vi "GetXPos.vi"(7 "Menu":refnum<class "Menu.lvclass">, 9 "SubMenu":bool[](array[boolean]), 10 "Array":T1[](array[typedef]), 11 "Item Names":string[](array[string])) -> (1 "ShortCut Text":string[](array[string]), 2 "Start ShortCut":i16, 3 "Total X":i16)   [LabVIEW 2021, in "Menu.lvlib" / "Menu.lvclass"]
uses:
  Menu.lvclass
  <vilib>/Utility/miscctls.llb/LVMenuShortCut.ctl
  Picture2D/src/Text/Text.lvclass
  C:/GitHub/Picture2D/src/IDrawable/IDrawable.lvclass
  C:/GitHub/Picture2D/src/Picture2D/Picture2D.lvclass
  Picture2D/src/2DPictureControl/2DPictureControl.lvclass
  Picture2D/src/Color/Color.lvclass
  Picture2D/src/Collection/Collection.lvclass
  Picture2D/src/Point/Point.lvclass
  GetFont.vi
  GetDesiredFont.vi
  Picture2D/src/Font/Font.lvclass
panel:
  out "2D Picture out":picture
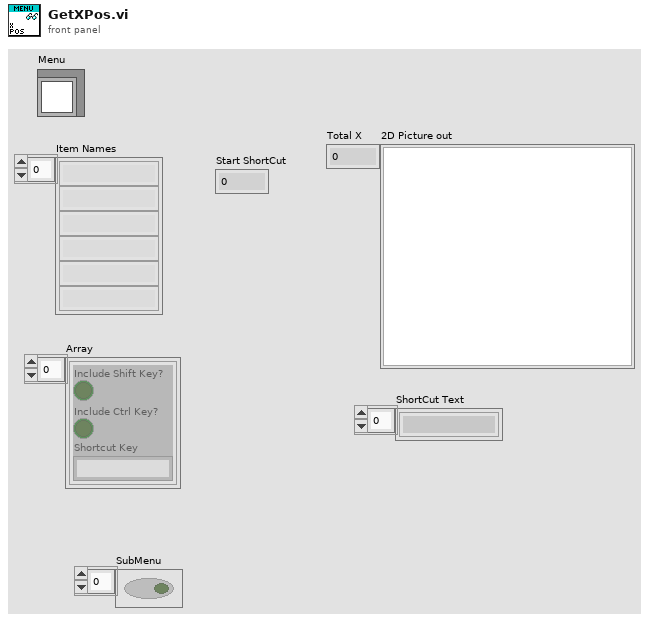
[diagram p1: front panel]
types:
  T1 = typedef "LVMenuShortCut.ctl" = cluster{"Include Shift Key?":bool, "Include Ctrl Key?":bool, "Shortcut Key":string}
  T2 = enum16{"User-specified Font", "Application Font", "System Font", "Dialog Font"}
  T3 = cluster{"left":i16, "top":i16, "right":i16, "bottom":i16}
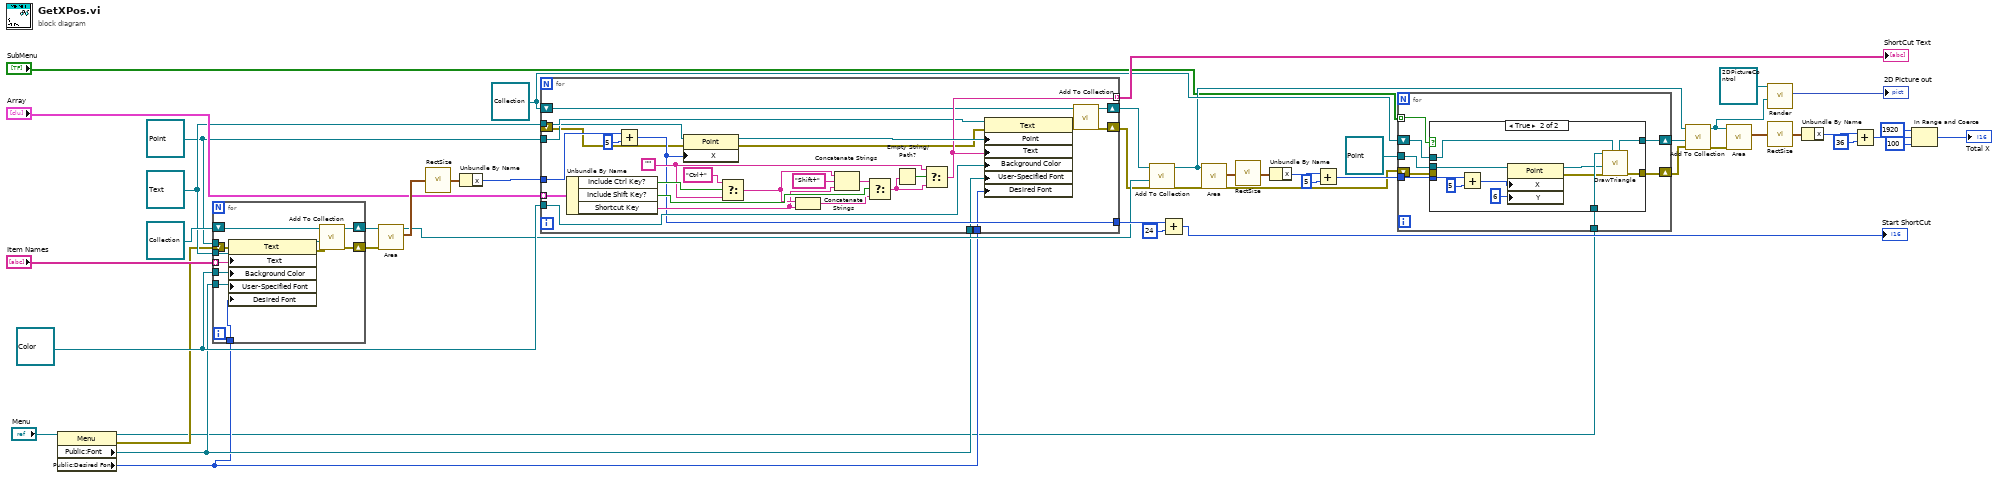
[diagram p0: block diagram]
diagram:
  w27 = refnum<class "Collection.lvclass"> refnum ("Picture2D.lvlib:Collection.lvclass")
  w34 = refnum<class "Color.lvclass"> refnum ("Color")
  w35 = refnum<class "Point.lvclass"> refnum ("Point")
  w36 = refnum<class "Text.lvclass"> refnum ("Text in")
  n1 = property class="Menu"(reference="Menu") -> (reference out=w1:refnum<class "Menu.lvclass">, error out=w2:errorcluster, "Public:Font"=w4:refnum<class "Font.lvclass">, "Public:Desired Font"=w3:T2)  [unwired: 1 in]
  n2 = for {
    tunnel: w36 -> [w56]
    tunnel: "Item Names" -> [w57] mode=indexing
    shift-right: [w58] -> w46
    shift-left: refnum<class "Collection.lvclass"> refnum ("Picture2D.lvlib:Collection.lvclass") -> [w59]
    tunnel: w35 -> [_]
    tunnel: w34 -> [w54]
    tunnel: w4 -> [w53]
    tunnel: w3 -> [w52]
    shift-right: [w50] -> w6
    shift-left: w2 -> [w49]
    n3 = property class="Text"(reference=w56, error in=w49, "Text"=w57, "Background Color"=w54, "User-Specified Font"=w53, "Desired Font"=w52) -> (reference out=w55:refnum<class "Text.lvclass">, error out=w51:errorcluster)
    n4 = call-dynamic "Add To Collection.vi"("error in (no error)"=w51, "IDrawable"=w55, "Collection in"=w59) -> ("error out"=w50:errorcluster, "Collection out"=w58:refnum<class "Collection.lvclass">)  [unwired: 7 in]
  }
  n5 = call-dynamic "Area.vi"("error in (no error)"=w6, "Collection in"=w46) -> ("Area"=w47:T3, "Collection out"=w29:refnum<class "Collection.lvclass">)  [unwired: 7 in, 1 out]
  n6 = call <vilib>:"RectSize.vi"("rect"=w47) -> ("point"=w48:cluster{"x":i16, "y":i16})
  n7 = Unbundle By Name(w48) -> ("x"=w33:i16)
  n8 = for {
    tunnel: "Array" -> [w82] mode=indexing
    shift-right: [w79] -> w28
    shift-left: w27 -> [w65]
    tunnel: [w72] -> w38 mode=indexing
    tunnel: w36 -> [w71]
    tunnel: w35 -> [w70]
    tunnel: w33 -> [w69]
    tunnel: w34 -> [w68]
    tunnel: [w66] -> w32
    tunnel: w4 -> [w64]
    tunnel: w3 -> [w63]
    shift-right: [w62] -> w7
    shift-left: _ -> [w61]
    w77 = ""
    n9 = Unbundle By Name(w82) -> ("Include Ctrl Key?"=w86:bool, "Include Shift Key?"=w87:bool, "Shortcut Key"=w74:string)
    n10 = Add(x=w69, y=i16 5) -> (x+y=w66:i16)
    n11 = property class="Point"(reference=w70, error in=w61, "X"=w66) -> (reference out=w80:refnum<class "Point.lvclass">, error out=w60:errorcluster)
    n12 = Select(t="Ctrl+" ("f"), s=w86, f=w77) -> (s? t:f=w75:string)
    n13 = Concatenate Strings(w75, w74) -> (w73:string)
    n14 = Concatenate Strings(w75, "Shift+" ("f"), w74) -> (w83:string)
    n15 = Select(t=w83, s=w87, f=w73) -> (s? t:f=w76:string)
    n16 = Empty String/Path?(string/path=w76) -> (empty?=w78:bool)
    n17 = Select(t=w77, s=w78, f=w76) -> (s? t:f=w72:string)
    n18 = property class="Text"(reference=w71, error in=w60, "Point"=w80, "Text"=w72, "Background Color"=w68, "User-Specified Font"=w64, "Desired Font"=w63) -> (reference out=w81:refnum<class "Text.lvclass">)  [unwired: 1 out]
    n19 = call-dynamic "Add To Collection.vi"("IDrawable"=w81, "Collection in"=w65) -> ("error out"=w62:errorcluster, "Collection out"=w79:refnum<class "Collection.lvclass">)  [unwired: 8 in]
  }
  "ShortCut Text" <- w38
  n20 = call-dynamic "Add To Collection.vi"("error in (no error)"=w7, "IDrawable"=w29, "Collection in"=w28) -> ("error out"=w8:errorcluster, "Collection out"=w23:refnum<class "Collection.lvclass">)  [unwired: 7 in]
  n21 = Add(x=w32, y=i16 24) -> (x+y=→"Start ShortCut":i16)
  n22 = call-dynamic "Area.vi"("error in (no error)"=w8, "Collection in"=w23) -> ("error out"=w9:errorcluster, "Area"=w44:T3)  [unwired: 7 in, 1 out]
  n23 = call <vilib>:"RectSize.vi"("rect"=w44) -> ("point"=w43:cluster{"x":i16, "y":i16})
  n24 = Unbundle By Name(w43) -> ("x"=w40:i16)
  n25 = Add(x=w40, y=i16 5) -> (x+y=w25:i16)
  n26 = for {
    shift-right: [w95] -> w24
    shift-left: w27 -> [w94]
    tunnel: refnum<class "Point.lvclass"> refnum ("Point") -> [w93]
    tunnel: w25 -> [w92]
    tunnel: "SubMenu" -> [w91] mode=indexing
    tunnel: w1 -> [w90]
    shift-right: [w89] -> w11
    shift-left: w9 -> [w88]
    n27 = case shown="True" w91 {
      tunnel: [w97 w101] -> w95
      tunnel: w94 -> [w97 w102]
      tunnel: w93 -> [_ w108]
      tunnel: w92 -> [_ w107]
      tunnel: w90 -> [_ w103]
      tunnel: [w96 w98] -> w89
      tunnel: w88 -> [w96 _]
      frame False {
      }
      frame True {
        n28 = Add(x=w107, y=i16 5) -> (x+y=w106:i16)
        n29 = property class="Point"(reference=w108, "X"=w106, "Y"=i16 6 ("Point:y")) -> (reference out=w100:refnum<class "Point.lvclass">, error out=w99:errorcluster)  [unwired: 1 in]
        n30 = call "DrawTriangle.vi"("Collection in"=w102, "error in"=w99, "Point"=w100, "Menu in"=w103) -> ("error out"=w98:errorcluster, "Collection out"=w101:refnum<class "Collection.lvclass">)  [unwired: 5 in, 1 out]
      }
    }
  }
  n31 = call-dynamic "Add To Collection.vi"("error in (no error)"=w11, "IDrawable"=w24, "Collection in"=w23) -> ("error out"=w10:errorcluster, "Collection out"=w20:refnum<class "Collection.lvclass">)  [unwired: 7 in]
  n32 = call-dynamic "Area.vi"("error in (no error)"=w10, "Collection in"=w20) -> ("Area"=w18:T3)  [unwired: 7 in, 2 out]
  n33 = call-dynamic "Render.vi"("IDrawable"=w20, "2DPictureControl in"=refnum<class "2DPictureControl.lvclass"> refnum) -> ("2D Picture out"=→"2D Picture out":picture)  [unwired: 7 in, 2 out]
  n34 = call <vilib>:"RectSize.vi"("rect"=w18) -> ("point"=w19:cluster{"x":i16, "y":i16})
  n35 = Unbundle By Name(w19) -> ("x"=w17:i16)
  n36 = Add(x=w17, y=i16 36) -> (x+y=w16:i16)
  n37 = In Range and Coerce(upper limit=i16 1920, x=w16, lower limit=i16 100) -> (coerced(x)=→"Total X":i16)  [unwired: 1 out]
